vi "RDV-handle-Filter.vi"(7 "Lower Cut-Off":dbl=30000.0 format="%#_13g", 8 "error in (no error)":errorcluster, 11 "RDV-Reflection_Data_viewer in":refnum<class "RDV-Reflection_Data_viewer.lvclass">) -> (0 "error out":errorcluster, 3 "RDV-Reflection_Data_viewer out":refnum<class "RDV-Reflection_Data_viewer.lvclass">)   [LabVIEW 2020, in "RDV-Reflection_Data_viewer.lvclass"]
doc: "Filters all data in the viewer's map with RDC-filter_box at the lower cut-off and adds the results to the map."
uses:
  RDV-Reflection_Data_viewer.lvclass
  Computation/RDC-Reflection_Data_Computation.lvlib
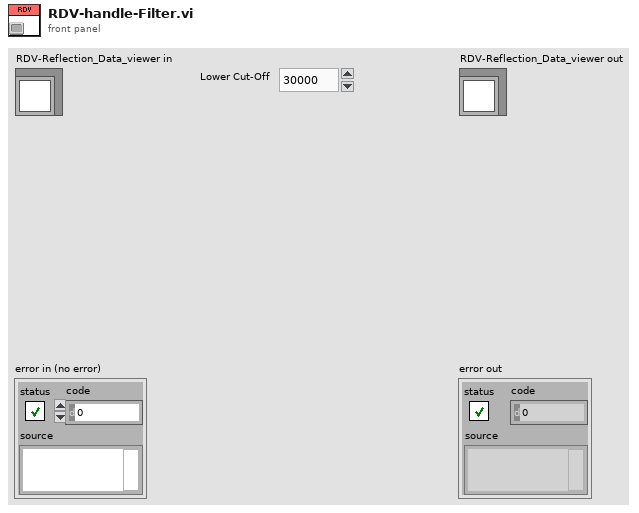
[diagram p1: front panel]
types:
  T1 = typedef "RFH-Reflection_File_Handler.lvlib/RFH-common_data_format.ctl" = cluster{"Frequency":dbl[], "Reflection'":dbl[], "Reflection''":dbl[], "Permativity'":dbl[], "Permativity''":dbl[], "Conductivity":dbl[], "Loss Tangent":dbl[], "Resistance":dbl[], "Reactance":dbl[]}
  T2 = typedef "RDV-Reflection_Data_viewer.lvclass/RDV-DATA_MAP_CLUST.ctl" = cluster{"filename w/ ext":string, "Common Format":T1}
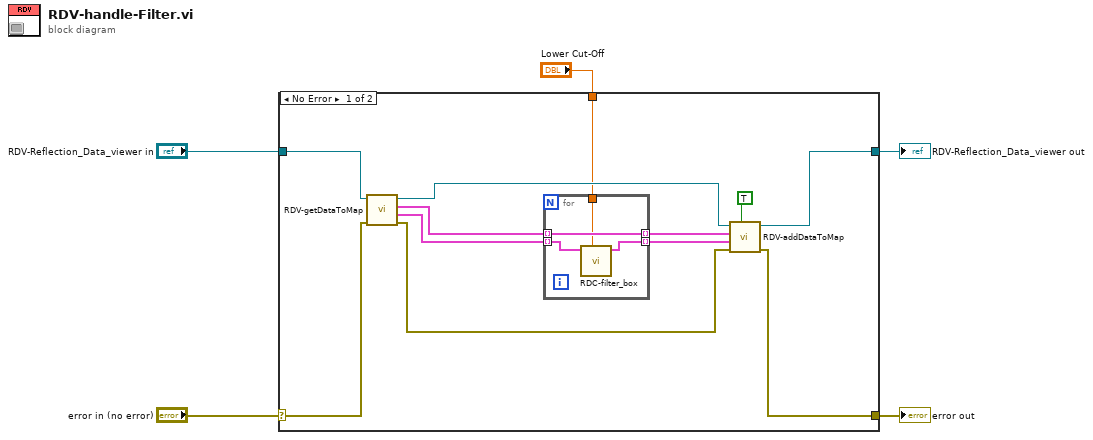
[diagram p0: block diagram]
diagram:
  n1 = case shown="No Error" "error in (no error)" {
    selector: "error in (no error)" -> [w7 w23]
    tunnel: [w8 w23] -> w4
    tunnel: [w9 w22] -> w2
    tunnel: "RDV-Reflection_Data_viewer in" -> [w10 w22]
    tunnel: "Lower Cut-Off" -> [w6 _]
    frame No Error {
      n2 = call "RDV-getDataToMap.vi"("error in (no error)"=w7, "RDV-Reflection_Data_viewer in"=w10) -> ("error out"=w15:errorcluster, "data"=w16:T1[], "all data"=w17:cluster{"key":string, "data":T2}[], "RDV-Reflection_Data_viewer out"=w11:refnum<class "RDV-Reflection_Data_viewer.lvclass">)  [unwired: 6 in]
      n3 = for {
        tunnel: w17 -> [w21] mode=indexing
        tunnel: w16 -> [w20] mode=indexing
        tunnel: [w19] -> w13 mode=indexing
        tunnel: [w21] -> w14 mode=indexing
        tunnel: w6 -> [w18]
        n4 = call "RDC-filter_box.vi"("Lower Cut-Off"=w18, "input cluster"=w20) -> ("output cluster"=w19:T1)  [unwired: 9 in]
      }
      n5 = call "RDV-addDataToMap.vi"("Use ignore list (false)"=TRUE, "error in (no error)"=w15, "data"=w13, "all data"=w14, "RDV-Reflection_Data_viewer in"=w11) -> ("error out"=w8:errorcluster, "RDV-Reflection_Data_viewer out"=w9:refnum<class "RDV-Reflection_Data_viewer.lvclass">)  [unwired: 5 in]
    }
    frame Error {
    }
  }
  "error out" <- w4
  "RDV-Reflection_Data_viewer out" <- w2
